vi "Get Menu Action.vi"(8 "error in":errorcluster, 9 "Button Index":i32=-1, 10 "Right Side?":bool, 11 "Menu":T2) -> (0 "error out":errorcluster, 3 "Action":T1=enum."None")   [LabVIEW 2026]
doc: "Looks up which state the ATM state machine must run when a function button is pressed. Takes the menu currently shown (ATM Menu.ctl), the side the button is on (Right Side?) and its Button Index, and returns the Action of that menu item. A Button Index outside 0..2 (for example -1 from Get Pressed Button Index.vi when nothing is pressed) returns None.\n\nError behaviour: error in is passed to error out unchanged; the action is computed in every case."
uses:
  Controls/ATM States.ctl
  Controls/ATM Menu Item.ctl
  Controls/ATM Menu Side.ctl
  Controls/ATM Menu.ctl
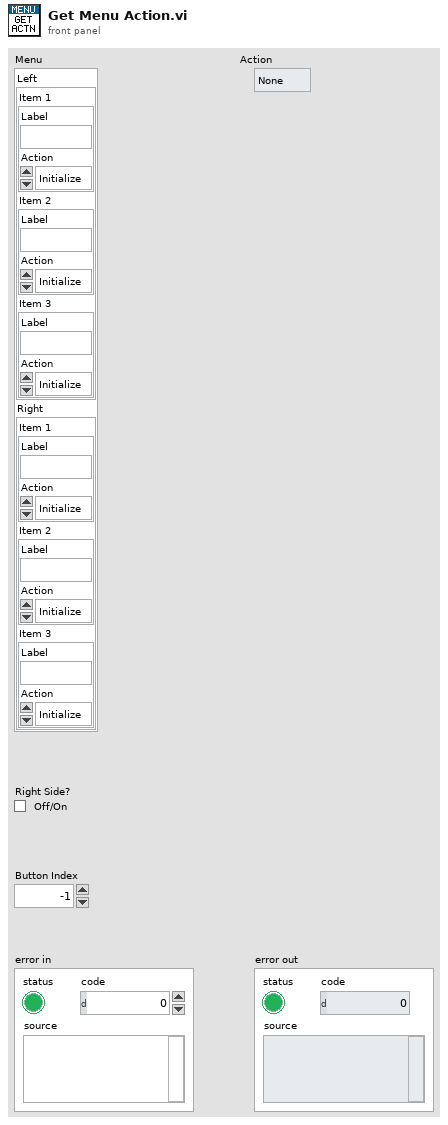
[diagram p1: front panel]
types:
  T1 = typedef "ATM States.ctl" = enum16{"Initialize", "Wait for Event", "Card Inserted", "Process Input", "Verify Account", "Show Main Menu", "Deposit Prompt", "Withdraw Prompt", "Deposit", "Withdraw", "Fast Cash", "Balance Inquiry", "None", "Terminate Session", "Exit"}
  T2 = typedef "ATM Menu.ctl" = cluster{"Left":T3, "Right":T3}
  T3 = typedef "ATM Menu Side.ctl" = cluster{"Item 1":T4, "Item 2":T4, "Item 3":T4}
  T4 = typedef "ATM Menu Item.ctl" = cluster{"Label":string, "Action":T1}
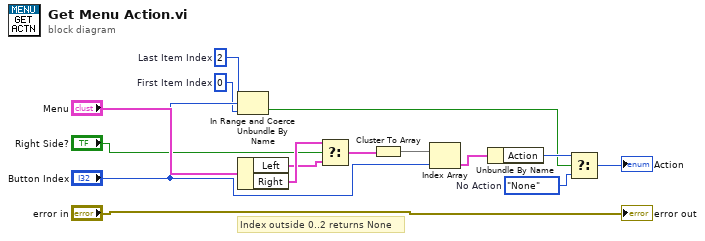
[diagram p0: block diagram]
diagram:
  w3 = ATM_States."None"  # No Action
  w6 = 0  # First Item Index
  w8 = 2  # Last Item Index
  # "Index outside 0..2 returns None"
  n1 = In Range and Coerce(upper limit=w8, x="Button Index", lower limit=w6) -> (In Range?=w4:bool)  [unwired: 1 out]
  n2 = Unbundle By Name("Menu") -> ("Left"=w12:T3, "Right"=w14:T3)
  n3 = Select(t=w14, s="Right Side?", f=w12) -> (s? t:f=w11:T3)
  n4 = Cluster To Array(cluster=w11) -> (array=w10:T4[])
  n5 = Index Array(array=w10, index="Button Index") -> (element=w9:T4)
  n6 = Unbundle By Name(w9) -> ("Action"=w5:T1)
  n7 = Select(t=w5, s=w4, f=w3) -> (s? t:f=→"Action":T1)
  "error out" <- "error in"
